vi "Process.vi"(8 "error in":errorcluster, 11 "LHF.SimpleAuth.User":refnum<class "LHF.SimpleAuth.User.lvclass">) -> (0 "error out":errorcluster={"status"=TRUE, "code"=1556, "source"="In Place Element Structure in SMO.lvclass:GetProtectedEvents.vi->SMO.lvclass:Process.vi:5310001->SMO.UI.lvclass:Process.vi:5310001->LHF.SimpleAuth.User.lvclass:Process.vi"}, 3 "LHF.SimpleAuth.User out":refnum<class "LHF.SimpleAuth.User.lvclass">)   [LabVIEW 2013, in "LHF.SimpleAuth.User.lvclass"]
doc: "---------------------------------------------------------------\nJKI State Machine Objects™\nhttp://jki.net/state-machine-objects/\nCopyright (C) 2005-2015, JKI <info@jki.net>\nALL RIGHTS RESERVEDJKI State Machine Objects (SMO) 1.0.0.5\nJKI - JKI\nCopyright (c) 2016, JKI"
uses:
  LHF.SimpleAuth.User.lvclass
  <vilib>/JKI/JKI SMO/SMO/Typedefs/Parent Call--Enum.ctl
  <vilib>/JKI/JKI SMO/SMO.UI/SMO.UI.lvclass
  src/LHF.DB.Mongo.lvclass
  <userlib>/_OpenG.lib/md5/md5.llb/MD5 Message Digest (Hexadecimal String)__ogtk.vi
  <vilib>/JKI/JKI SMO/SMO/SMO.lvclass
panel:
  in  "Action: Edit >> Level":T1(ring)
  in  "Action: Edit >> Name":string
  in  "Action: Edit >> Login":string
  in  "Action: Load User":i32(listbox)=-1
  in  "Action: Search":string
  in  "Action: Save":bool
  in  "Action: Set Password":bool
  in  "Action: Remove":bool
  # "For instructions on how to use the JKI State Machine Objects, examples and video tutorials, visit:\nhttp://jki.net/state-machine-objects/\n\nJKI State Machine Objects™\nhttp://jki.net/state-machine-objects/\nCopyright (C) 2005-2015, JKI <info@jki.net>\nALL RIGHTS RESERVED"
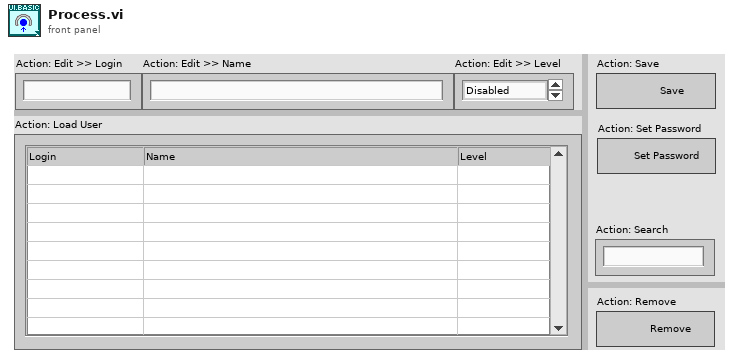
[diagram p1: front panel]
types:
  T1 = enum16{"Disabled", "Operator", "Engineer", "Administrator"}
  T2 = typedef "SMO.lvclass/Parent Call--Enum.ctl" = enum16{"Allows parent to run", "Does not request parent to run"}
  T3 = enum32{"invalid app kind", "Development System", "Run Time System", "Student Edition", "Embedded LabVIEW", "Evaluation", "Custom"}
  T4 = enum32{"Invalid", "Standard", "Closed", "Hidden", "Minimized", "Maximized"}
  T5 = enum32{"Bad", "Idle", "Run top level", "Running"}
  T6 = cluster{"Core":cluster{"Current VI Reference":refnum<vi>, "Close Panel on Exit?":bool, "error":errorcluster}, "Self Reference":refnum<class "LHF.SimpleAuth.User.lvclass">, "Mongo":refnum<class "LHF.DB.Mongo.lvclass">, "_id Array":string[], "_id":string, "User":cluster{"login":string, "name":string, "level":u8}, "Edit":cluster{"login":string, "name":string, "level":u8}}
  T7 = cluster{"login":string, "name":string, "level":u8}
  T8 = cluster{"Current VI Reference":refnum<vi>, "Close Panel on Exit?":bool, "error":errorcluster}
  T9 = typedef "SMO.lvclass/Protected Events.ctl" = cluster{"StopProcesses":refnum<user-event>, "AbortProcesses":refnum<user-event>, "Config Changed":refnum<user-event>}
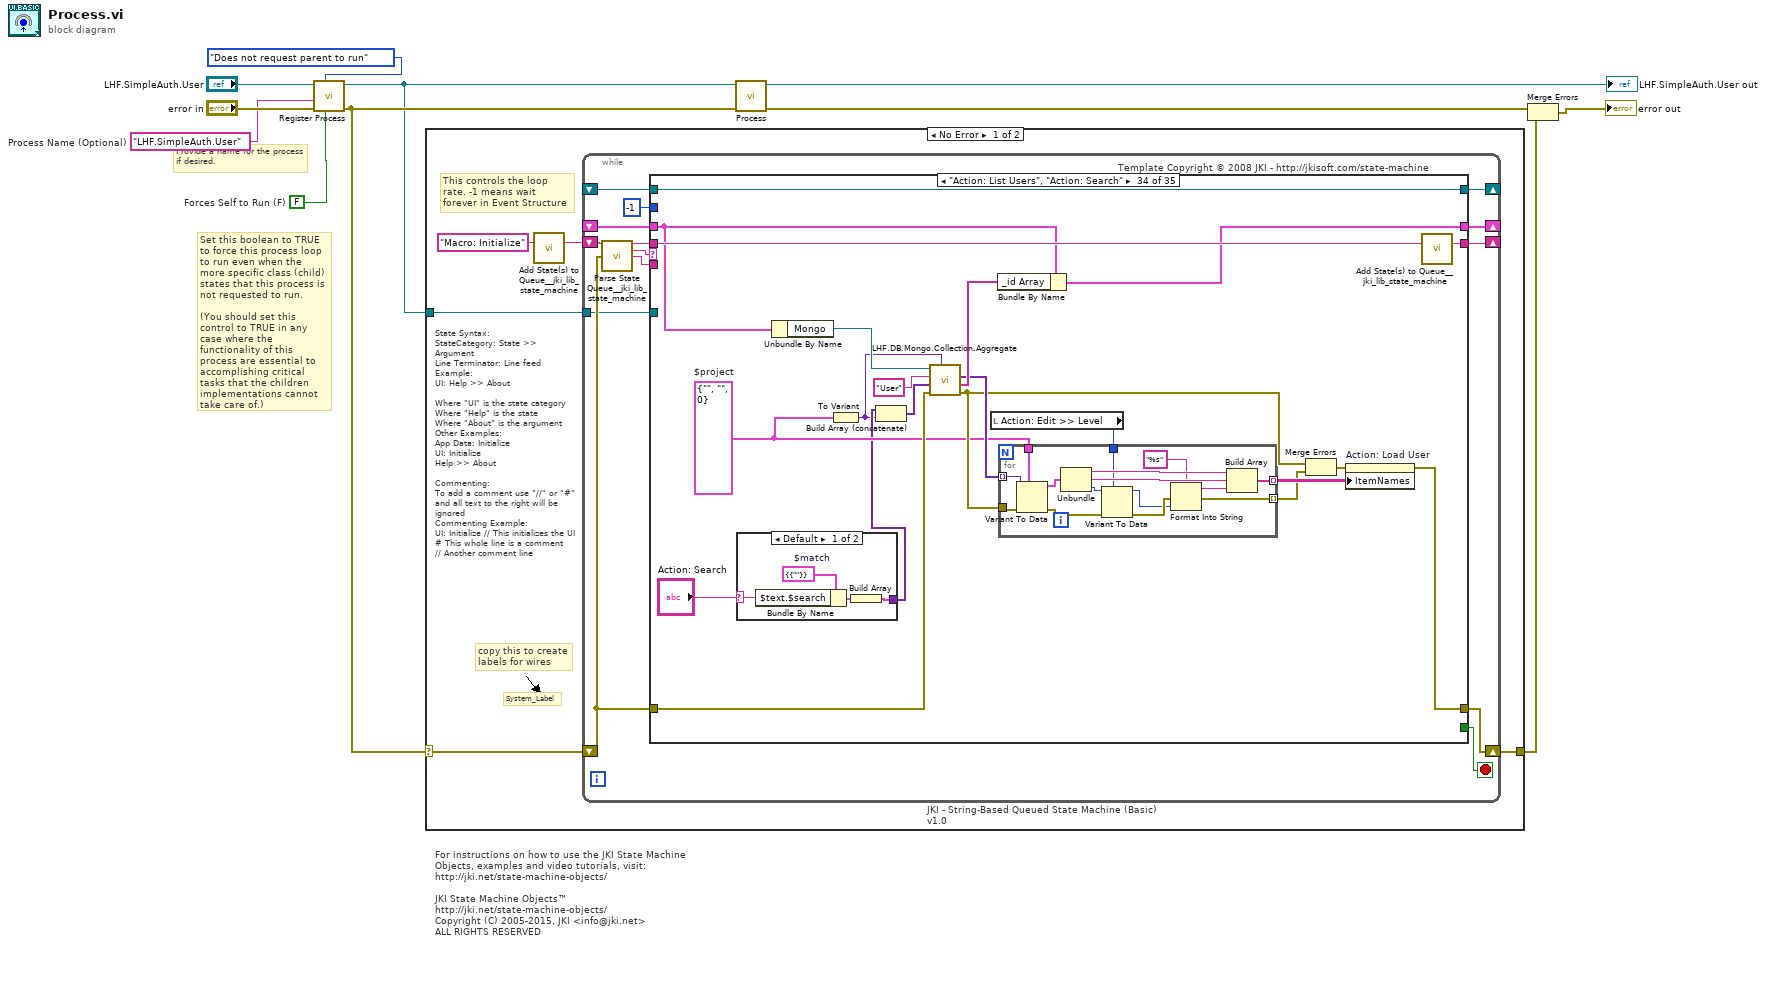
[diagram p0: block diagram]
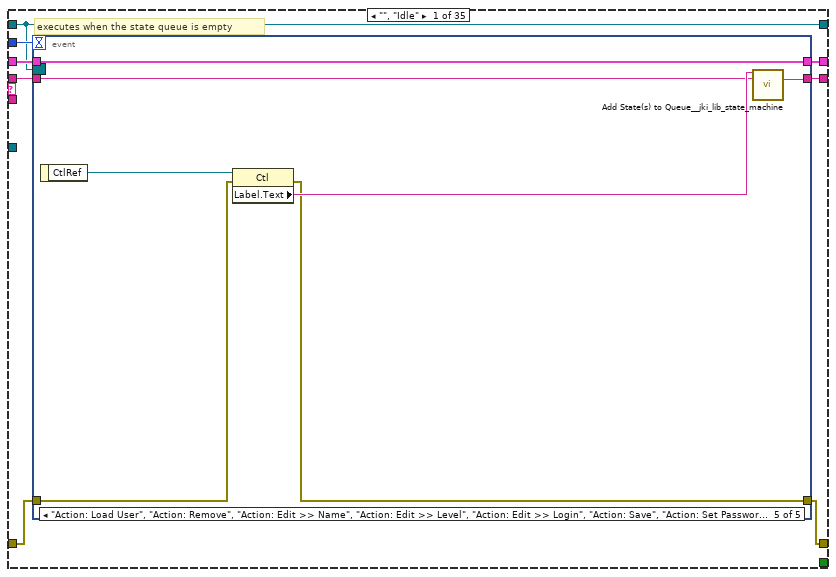
[diagram p2: hidden frame]
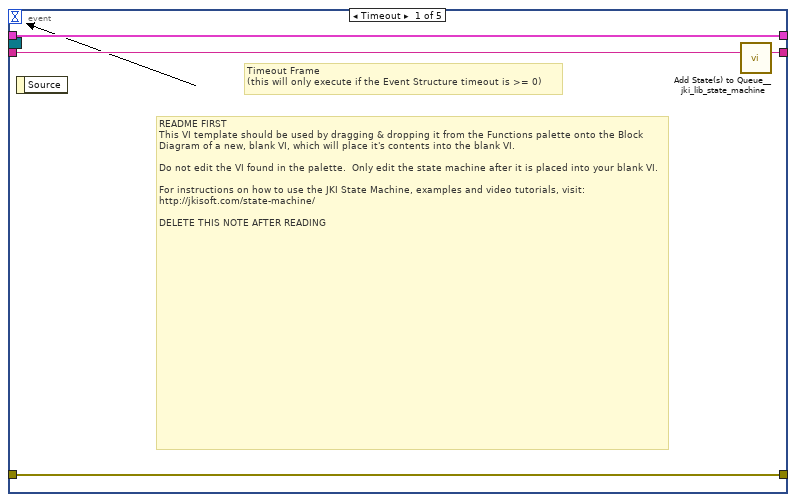
[diagram p3: hidden frame]
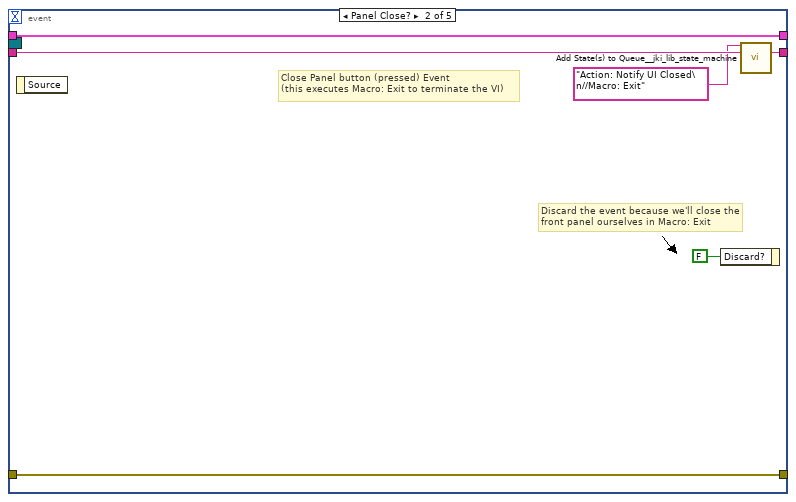
[diagram p4: hidden frame]
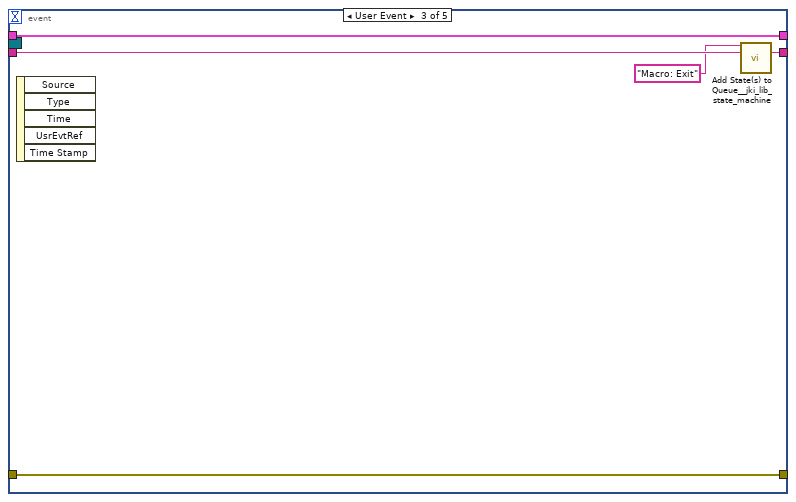
[diagram p5: hidden frame]
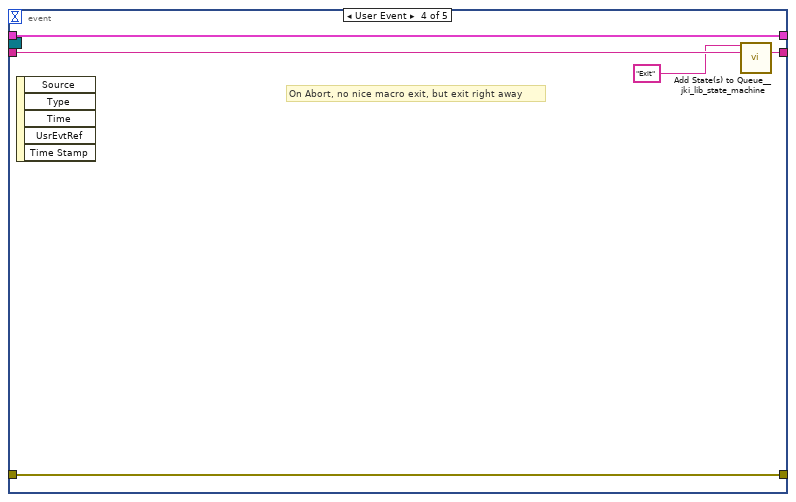
[diagram p6: hidden frame]
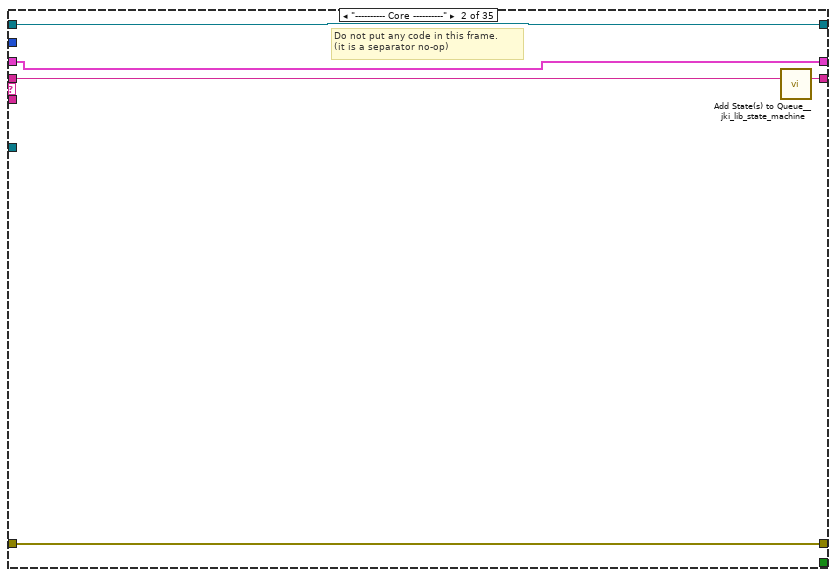
[diagram p7: hidden frame]
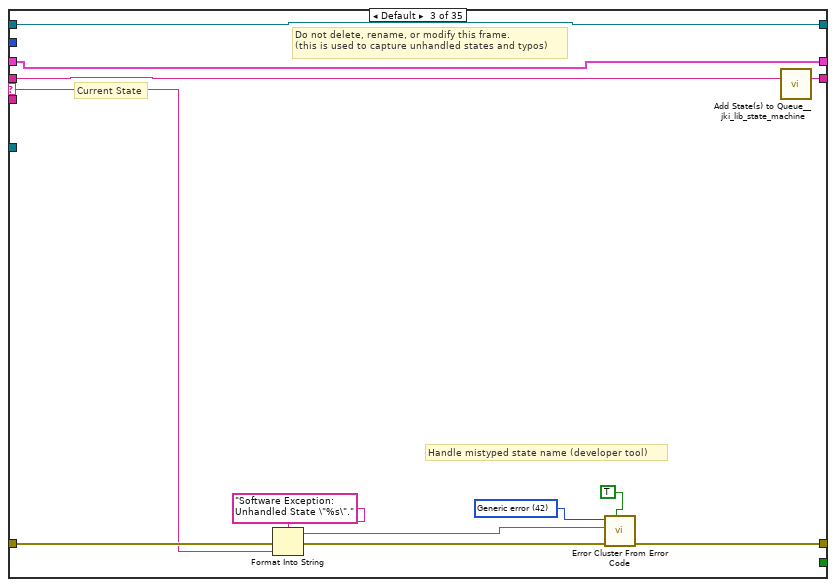
[diagram p8: hidden frame]
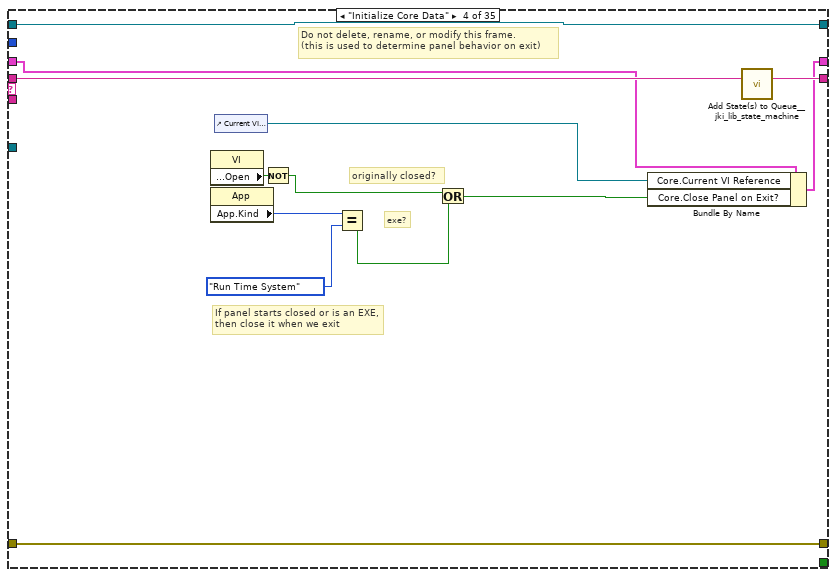
[diagram p9: hidden frame]
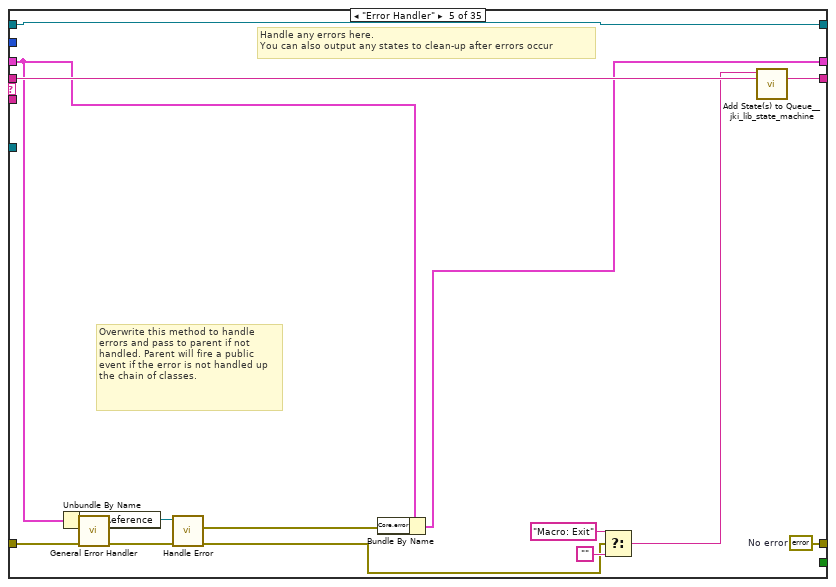
[diagram p10: hidden frame]
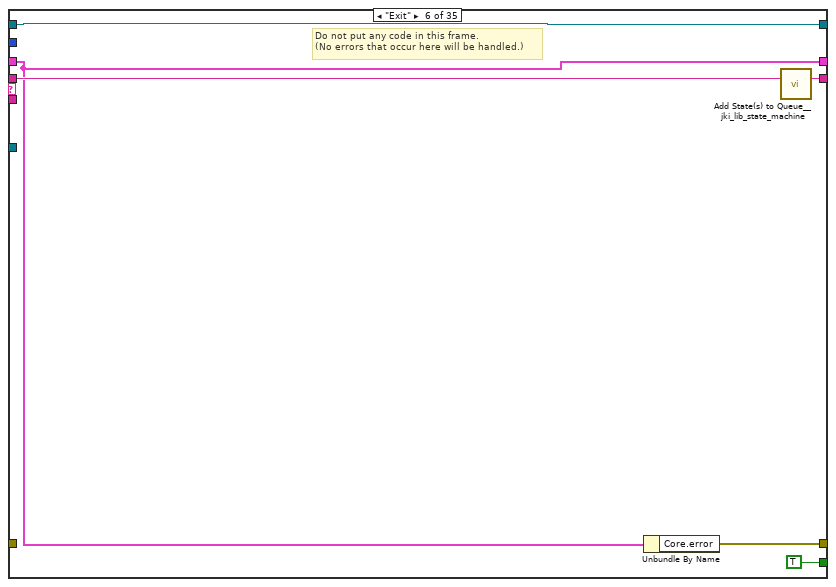
[diagram p11: hidden frame]
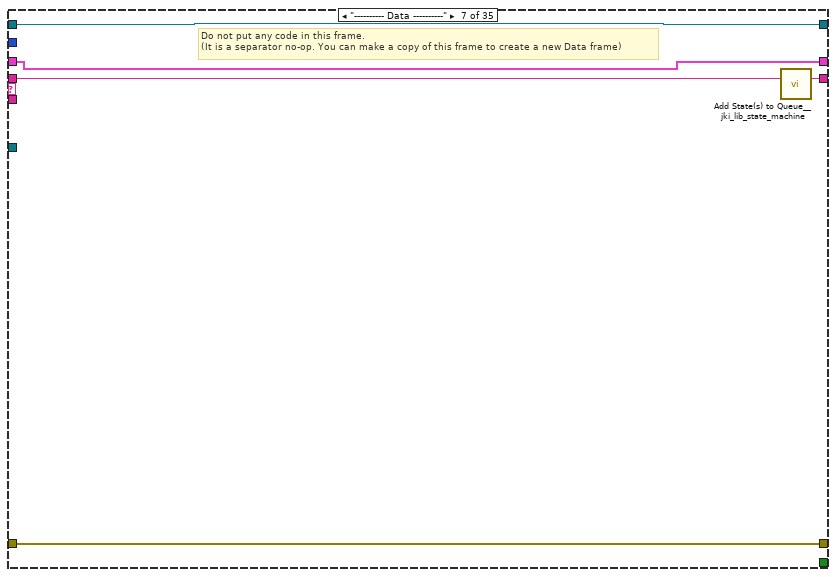
[diagram p12: hidden frame]
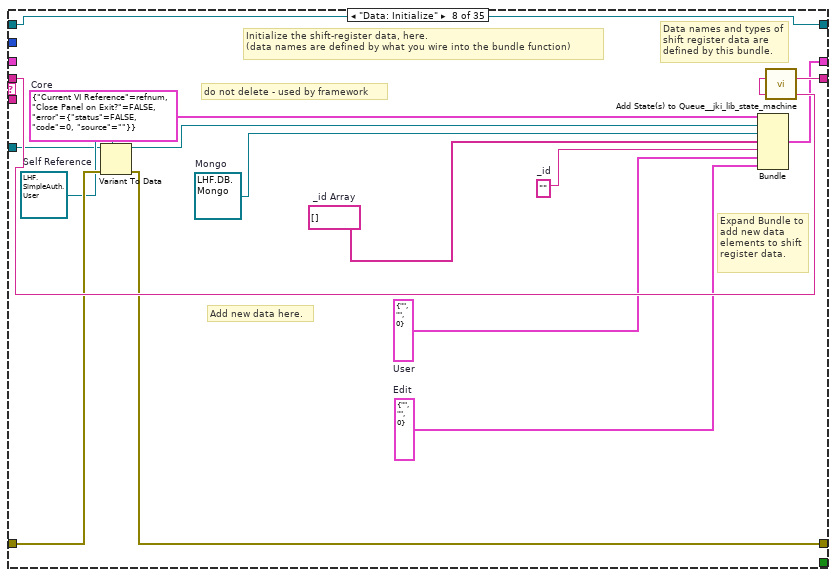
[diagram p13: hidden frame]
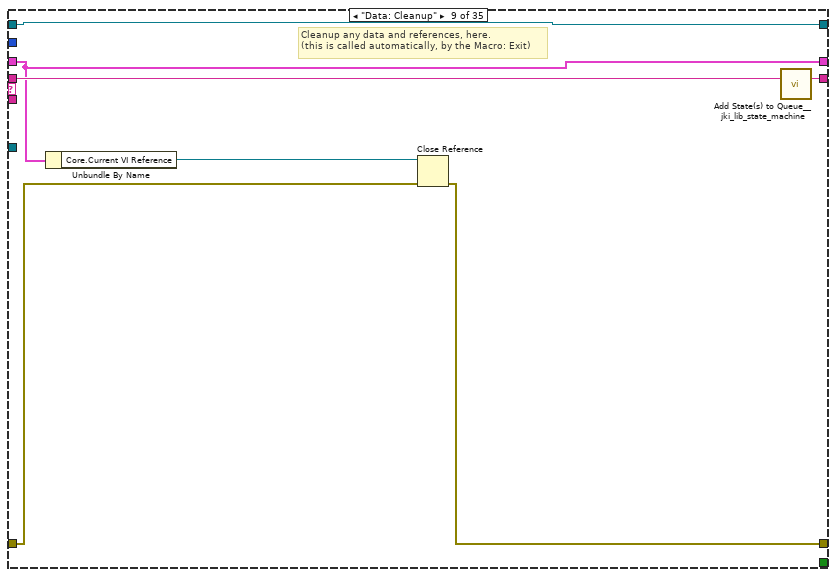
[diagram p14: hidden frame]
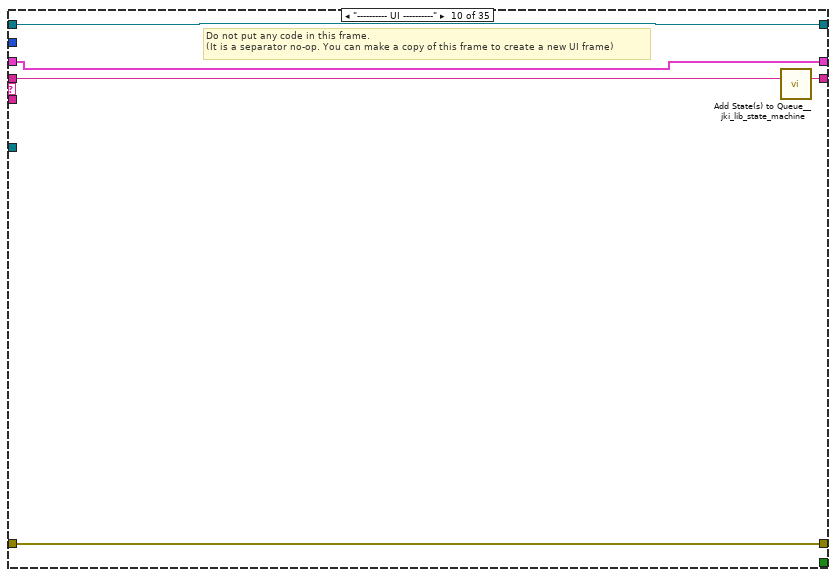
[diagram p15: hidden frame]
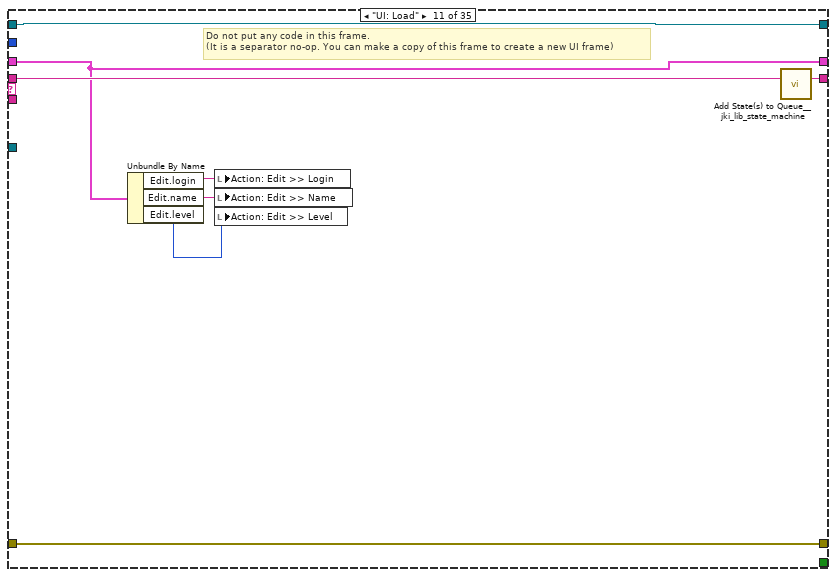
[diagram p16: hidden frame]
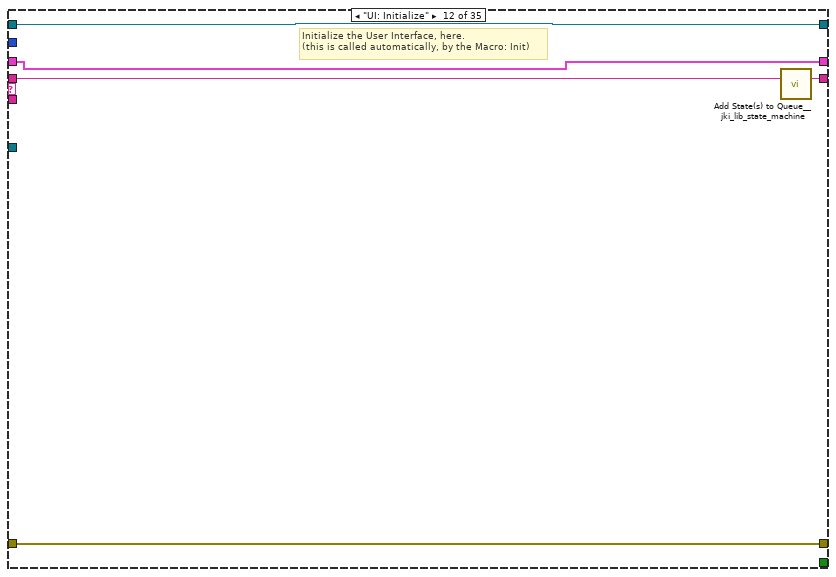
[diagram p17: hidden frame]
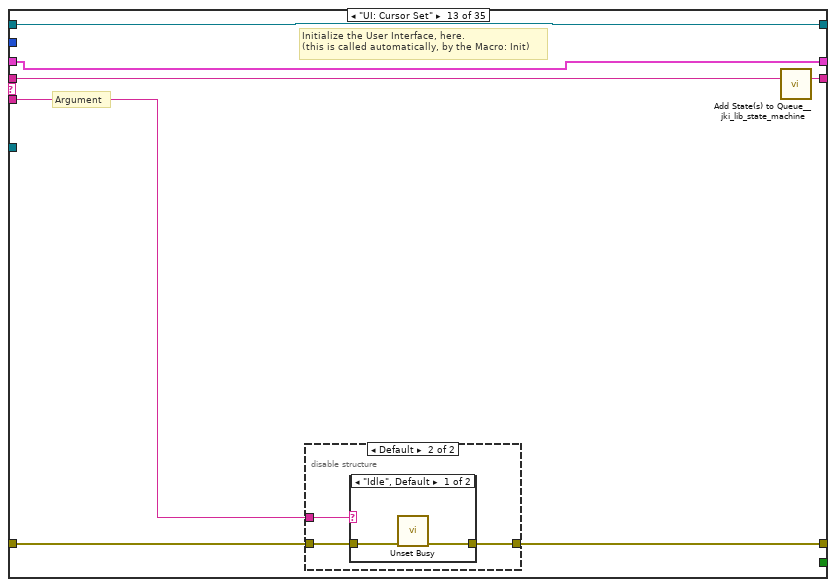
[diagram p18: hidden frame]
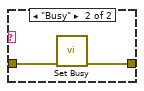
[diagram p20: hidden frame]
diagram:
  w2 = FALSE  # Forces Self to Run (F)
  w1 = "LHF.SimpleAuth.User"  # Process Name (Optional)
  # "Provide a name for the process\nif desired."
  # "Set this boolean to TRUE to force this process loop to run even when the more specific class (child) states that this process is not requested to run.\n\n(You should set this control to TRUE in any case where the functionality of this process are essential to accomplishing critical tasks that the children implementations cannot take care of.)"
  # "For instructions on how to use the JKI State Machine Objects, examples and video tutorials, visit:\nhttp://jki.net/state-machine-objects/\n\nJKI State Machine Objects™\nhttp://jki.net/state-machine-objects/\nCopyright (C) 2005-2015, JKI <info@jki.net>\nALL RIGHTS RESERVED"
  n1 = call <vilib>:"Register Process.vi"("Forces Self to Run (F)"=w2, "Parent Call"=Parent_Call--Enum."Does not request parent to run", "error in (no error)"="error in", "Process Name (optional)"=w1, "SMO"="LHF.SimpleAuth.User") -> ("error out"=w8:errorcluster, "SMO out"=w7:refnum<class "LHF.SimpleAuth.User.lvclass">)  [unwired: 5 in]
  n2 = case shown="No Error" w8 {
    selector: w8 -> [w13 w506]
    tunnel: w7 -> [w14 _]
    tunnel: [w12 w506] -> w4
    frame No Error {
      # "State Syntax:\nStateCategory: State >> Argument\nLine Terminator: Line feed\nExample:\nUI: Help >> About\n\nWhere \"UI\" is the state category\nWhere \"Help\" is the state\nWhere \"About\" is the argument\nOther Examples:\nApp Data: Initialize\nUI: Initialize\nHelp >> About\n\nCommenting:\nTo add a comment use \"//\" or \"#\" and all text to the right will be ignored\nCommenting Example:\nUI: Initialize // This initializes the UI\n# This whole line is a comment\n// Another comment line"
      # "copy this to create labels for wires"
      # "This controls the loop rate. -1 means wait forever in Event Structure"
      # "System_Label"
      n3 = call <vilib>:"Add State(s) to Queue__jki_lib_state_machine.vi"("State(s) in (\"\")"="Macro: Initialize") -> ("States Out"=w16:string)  [unwired: 14 in]
      n4 = while "JKI - String-Based Queued State Machine (Basic) v1.0" {
        shift-right: [w23] -> _
        shift-left: _ -> [w22]
        shift-right: [w26] -> w12
        shift-left: w13 -> [w20]
        shift-right: [w25] -> _
        shift-left: w16 -> [w27]
        tunnel: w14 -> [w19]
        shift-right: [w18] -> _
        shift-left: _ -> [w17]
        stop <- w24 stop-if-true
        # "Template Copyright © 2008 JKI - http://jkisoft.com/state-machine"
        n5 = call <vilib>:"Parse State Queue__jki_lib_state_machine.vi"("State Queue"=w27, "Error In (no error)"=w20) -> ("Remaining States"=w29:string, "Current State"=w30:string, "Arguments"=w28:string)  [unwired: 11 in]
        n6 = case shown="\"Action: List Users\", \"Action: Search\"" w30 {
          selector: w30 -> [_ _ w72 _ _ _ _ _ _ _ _ _ _ _ _ _ _ _ _ _ _ _ _ _ _ _ _ _ _ _ _ _ _ _ _]
          tunnel: w29 -> [w38 w70 w76 w95 w109 w115 w120 w135 w142 w147 w155 w160 w167 w183 w215 w229 w243 w248 w259 w264 w275 w290 w295 w304 w318 w341 w351 w361 w378 w410 w421 w430 w439 w478 w505]
          tunnel: w28 -> [_ _ _ _ _ _ _ _ _ _ _ _ w161 w177 _ _ _ _ _ _ _ _ _ _ _ _ _ _ _ _ _ _ _ _ _]
          tunnel: w22 -> [w36 w67 w74 w86 w98 w111 w117 _ w137 w144 w148 w158 w165 w179 w212 w225 w234 w245 w256 w261 w273 w288 w293 w300 w315 w338 w349 w358 w375 w408 w418 w428 w436 w475 w501]
          tunnel: [w35 w68 w78 w92 w100 w110 w118 w131 w138 w145 w153 w157 w162 w180 w213 w227 w241 w246 w250 w262 w271 w285 w291 w297 w308 w332 w347 w353 w370 w406 w415 w426 w434 w474 w499] -> w26
          tunnel: w20 -> [w34 w68 w77 w92 w105 _ w118 w132 w139 w145 w153 w157 w163 w181 w213 w227 w241 w246 w251 w262 w272 w286 w291 w298 w309 w335 w347 w354 w371 w406 w413 w426 w435 w473 w500]
          tunnel: [w37 w69 w75 w94 w108 w114 w119 w134 w141 w146 w154 w159 w166 w182 w214 w228 w242 w247 w258 w263 w274 w289 w294 w303 w317 w340 w350 w360 w377 w409 w420 w429 w438 w477 w504] -> w25
          tunnel: [_ _ _ _ _ TRUE _ _ _ _ _ _ _ _ _ _ _ _ _ _ _ _ _ _ _ _ _ _ _ _ _ _ _ _ _] -> w24
          tunnel: [w33 w67 w74 w93 w97 w111 w117 w133 w137 w144 w148 w158 w165 w179 w212 w225 w234 w245 w256 w261 w273 w288 w293 w300 w307 w334 w349 w358 w375 w405 w418 w425 w433 w472 w501] -> w23
          tunnel: -1 ("Timeout") -> [w32 _ _ _ _ _ _ _ _ _ _ _ _ _ _ _ _ _ _ _ _ _ _ _ _ _ _ _ _ _ _ _ _ _ _]
          tunnel: w19 -> [_ _ _ _ _ _ _ w129 _ _ _ _ _ _ _ _ _ _ _ _ _ _ _ _ _ _ _ _ _ _ _ _ _ _ _]
          tunnel: [w31 w66 w71 w83 w107 w112 w116 w127 w136 w143 w152 w156 w164 w176 w211 w226 w235 w244 w257 w260 w270 w287 w292 w302 w316 w339 w348 w359 w376 w407 w419 w427 w437 w476 w503] -> w18
          tunnel: w17 -> [w31 w66 w71 w83 w107 w112 w116 w127 w136 w143 w152 w156 w164 w176 w211 w226 w235 w244 w257 w260 w266 w287 w292 w302 w316 w339 w348 w359 w376 w407 w419 w427 w437 w476 w503]
          frame "", "Idle" {
            # "executes when the state queue is empty"
            n7 = event shown="[4] \"Action: Load User\", \"Action: Remove\", \"Action: Edit >> Name\", \"Action: Edit >> Level\", \"Action: Edit >> Login\", \"Action: Save\", \"Action: Set Password\", \"Action: Search\": Value Change" {
              selector: w31 -> [_ _ _ _ _]
              dyn-events: _ -> [_ _ _ _ _]
              timeout: w32 -> [_ _ _ _ _]
              tunnel: w38 -> [w42 w48 w53 w58 w59]
              tunnel: [w41 w47 w52 w57 w64] -> w37
              tunnel: w36 -> [w39 w44 w50 w55 w60]
              tunnel: [w40 w43 w51 w56 w61] -> w35
              tunnel: w34 -> [w40 w43 w51 w56 w62]
              tunnel: [w39 w44 w50 w55 w60] -> w33
              event Timeout {
                # "README FIRST\nThis VI template should be used by dragging & dropping it from the Functions palette onto the Block Diagram of a new, blank VI, which will place it's contents into the blank VI.\n\nDo not edit the VI found in the palette.  Only edit the state machine after it is placed into your blank VI.\n\nFor instructions on how to use the JKI State Machine, examples and video tutorials, visit:\nhttp://jkisoft.com/state-machine/\n\nDELETE THIS NOTE AFTER READING"
                # "Timeout Frame\n(this will only execute if the Event Structure timeout is >= 0)"
                n8 = event-data() -> ()  [unwired: 1 in, 1 out]
                n9 = call <vilib>:"Add State(s) to Queue__jki_lib_state_machine.vi"("State(s) in (\"\")"=w42) -> ("States Out"=w41:string)  [unwired: 14 in]
              }
              event Panel Close? {
                # "Discard the event because we'll close the front panel ourselves in Macro: Exit"
                # "Close Panel button (pressed) Event\n(this executes Macro: Exit to terminate the VI)"
                n10 = event-data() -> ()  [unwired: 1 in, 1 out]
                n11 = event-data("Discard?"=FALSE) -> ()  [unwired: 1 in, 1 out]
                n12 = call <vilib>:"Add State(s) to Queue__jki_lib_state_machine.vi"("State(s) in Front (\"\")"="Action: Notify UI Closed\n//Macro: Exit", "State(s) in (\"\")"=w48) -> ("States Out"=w47:string)  [unwired: 13 in]
              }
              event User Event {
                n13 = event-data() -> ()  [unwired: 1 in, 5 out]
                n14 = call <vilib>:"Add State(s) to Queue__jki_lib_state_machine.vi"("State(s) in Front (\"\")"="Macro: Exit", "State(s) in (\"\")"=w53) -> ("States Out"=w52:string)  [unwired: 13 in]
              }
              event User Event {
                # "On Abort, no nice macro exit, but exit right away"
                n15 = event-data() -> ()  [unwired: 1 in, 5 out]
                n16 = call <vilib>:"Add State(s) to Queue__jki_lib_state_machine.vi"("State(s) in Front (\"\")"="Exit", "State(s) in (\"\")"=w58) -> ("States Out"=w57:string)  [unwired: 13 in]
              }
              event "Action: Load User", "Action: Remove", "Action: Edit >> Name", "Action: Edit >> Level", "Action: Edit >> Login", "Action: Save", "Action: Set Password", "Action: Search": Value Change {
                n17 = event-data() -> ("CtlRef"=w65:refnum<vi>)  [unwired: 1 in]
                n18 = property class="Ctl"(reference=w65, error in=w62) -> (error out=w61:errorcluster, "Label.Text"=w63:string)  [unwired: 1 out]
                n19 = call <vilib>:"Add State(s) to Queue__jki_lib_state_machine.vi"("State(s) in Front (\"\")"=w63, "State(s) in (\"\")"=w59) -> ("States Out"=w64:string)  [unwired: 13 in]
              }
            }
          }
          frame "---------- Core ----------" {
            # "Do not put any code in this frame.\n(it is a separator no-op)"
            n20 = call <vilib>:"Add State(s) to Queue__jki_lib_state_machine.vi"("State(s) in (\"\")"=w70) -> ("States Out"=w69:string)  [unwired: 14 in]
          }
          frame Default {
            w81 = 42 items=["No error", "Argument error", "Memory is full", "Out of zone", "End of file", "File already open", "Generic file I/O error", "File not found", "File permission error", "Disk is full", "Duplicate path", "Too many files open", "System feature not enabled", "Resource file not found", "Cannot add resource", "Resource not found", "Image not found", "Image memory error", "Pen does not exist", "Config type invalid", "Config token not found", "Config parse error", "Config memory error", "Bad external code format", "Bad external code offset", "External code not present", "Null window", "Destroy window error", "Null menu", "Print aborted", "Bad print record", "Print driver error", "Windows error during printing", "Memory error during printing", "Print dialog error", "Generic print error", "Invalid device refnum", "Device not found", "Device parameter error", "Device unit error", "Cannot open device", "Device call aborted", "Generic error", "Cancelled by user", "Object ID too low", "Object ID too high", "Object not in heap", "Unknown heap", "Unknown object (invalid DefProc)", "Unknown object (DefProc not in table)", "Message out of range", "Invalid (null) method", "Unknown message", "Manager call not supported", "Bad address", "Network operation in progress", "Network operation timed out", "Connection is busy", "Network attribute not supported", "Network error", "Address in use", "System out of memory", "Connection aborted", "Connection refused", "Not connected", "Already connected", "Connection closed", "Initialization error (interapplication manager)", "Bad occurrence", "Wait on unbound occurrence handler", "Occurrence queue overflow", "Datalog type conflict", "Unused", "Unrecognized type (interapplication manager)", "Memory corrupt", "Failed to make temporary DLL", "Old CIN version", "Drag socket not found", "Failed to load drop-object", "Failed to register OLE object", "Failed to release OLE object", "Format specifier type mismatch", "Unknown format specifier", "Too few format specifiers", "Too many format specifiers", "Scan failed", "Newer CIN version", "Error converting to variant", "Runtime menu error", "Password tampered", "Variant attribute not found", "Incompatible variant data type", "Event data is not available", "Event Store is not present", "Occurrence is not found", "Event Queue is not created", "Event info is not available", "Refnum passed is NULL", "Error retrieving Class GUID", "Error retrieving CoClass GUID", "Error retrieving TypeLib GUID.", "Bad built application magic bytes.", "Specific driver is different from the specific driver associated with the Logical Name.", "There is no session opened to the class driver.", "Max Error", "MAX - Error with config objects", "MAX - Error loading configuration", "MAX - Group not supported"]
            # "Current State"
            # "Do not delete, rename, or modify this frame.\n(this is used to capture unhandled states and typos)"
            # "Handle mistyped state name (developer tool)"
            n21 = Format Into String(format string="Software Exception: Unhandled State \"%s\"." ("message"), error in=w77, w72) -> (resulting string=w80:string, error out=w79:errorcluster)  [unwired: 1 in]
            n22 = call <vilib>:"Error Cluster From Error Code.vi"("show call chain? (False)"=TRUE, "error in (no error)"=w79, "error message (\"\")"=w80, "error code (0)"=w81) -> ("error out"=w78:errorcluster)  [unwired: 5 in]
            n23 = call <vilib>:"Add State(s) to Queue__jki_lib_state_machine.vi"("State(s) in (\"\")"=w76) -> ("States Out"=w75:string)  [unwired: 14 in]
          }
          frame "Initialize Core Data" {
            # "Do not delete, rename, or modify this frame.\n(this is used to determine panel behavior on exit)"
            # "originally closed?"
            # "exe?"
            # "If panel starts closed or is an EXE, then close it when we exit"
            n24 = property class="VI"() -> ("Front Panel.Open"=w91:bool)  [unwired: 2 in, 2 out]
            n25 = property class="App"() -> ("App.Kind"=w90:T3)  [unwired: 2 in, 2 out]
            n26 = control-ref of="Current VI Reference"() -> (w84:refnum<vi>)
            n27 = Not(x=w91) -> (.not. x?=w88:bool)
            n28 = Equal?(x=w90, y=T3."Run Time System" ("Application:Kind")) -> (x = y?=w87:bool)
            n29 = Or(x=w88, y=w87) -> (x .or. y?=w85:bool)
            n30 = Bundle By Name(cluster=w86, "Core.Current VI Reference"=w84, "Core.Close Panel on Exit?"=w85) -> (w93:T6)
            n31 = call <vilib>:"Add State(s) to Queue__jki_lib_state_machine.vi"("State(s) in (\"\")"=w95) -> ("States Out"=w94:string)  [unwired: 14 in]
          }
          frame "Error Handler" {
            w100 = errorcluster {"status"=FALSE, "code"=0, "source"=""}  # No error
            # "Overwrite this method to handle errors and pass to parent if not handled. Parent will fire a public event if the error is not handled up the chain of classes."
            # "Handle any errors here.\nYou can also output any states to clean-up after errors occur"
            n32 = Unbundle By Name(w98) -> ("Self Reference"=w106:refnum<class "LHF.SimpleAuth.User.lvclass">)
            n33 = call <vilib>:"General Error Handler.vi"("error in (no error)"=w105) -> ("error out"=w96:errorcluster)  [unwired: 10 in, 4 out]
            n34 = call-dynamic "Handle Error.vi"("error in"=w96, "SMO"=w106) -> ("handling error"=w101:errorcluster, "Unhandled error"=w99:errorcluster)  [unwired: 7 in, 1 out]
            n35 = Bundle By Name(cluster=w98, "Core.error"=w99) -> (w97:T6)
            n36 = Select(t="Macro: Exit", s=w101, f="") -> (s? t:f=w102:string)
            n37 = call <vilib>:"Add State(s) to Queue__jki_lib_state_machine.vi"("State(s) in Front (\"\")"=w102, "State(s) in (\"\")"=w109) -> ("States Out"=w108:string)  [unwired: 13 in]
          }
          frame "Exit" {
            # "Do not put any code in this frame.\n(No errors that occur here will be handled.)"
            n38 = Unbundle By Name(w111) -> ("Core.error"=w110:errorcluster)
            n39 = call <vilib>:"Add State(s) to Queue__jki_lib_state_machine.vi"("State(s) in (\"\")"=w115) -> ("States Out"=w114:string)  [unwired: 14 in]
          }
          frame "---------- Data ----------" {
            # "Do not put any code in this frame.\n(It is a separator no-op. You can make a copy of this frame to create a new Data frame)"
            n40 = call <vilib>:"Add State(s) to Queue__jki_lib_state_machine.vi"("State(s) in (\"\")"=w120) -> ("States Out"=w119:string)  [unwired: 14 in]
          }
          frame "Data: Initialize" {
            w121 = ""  # _id
            w122 = T7 {"login"="", "name"="", "level"=0}  # Edit
            w123 = T7 {"login"="", "name"="", "level"=0}  # User
            w124 = string[] []  # _id Array
            w125 = refnum<class "LHF.DB.Mongo.lvclass"> refnum  # Mongo
            w126 = T8 {"Current VI Reference"=refnum, "Close Panel on Exit?"=FALSE, "error"={"status"=FALSE, "code"=0, "source"=""}}  # Core
            w130 = refnum<class "LHF.SimpleAuth.User.lvclass"> refnum  # Self Reference
            # "do not delete - used by framework"
            # "Expand Bundle to add new data elements to shift register data."
            # "Add new data here."
            # "Data names and types of shift register data are defined by this bundle."
            # "Initialize the shift-register data, here.\n(data names are defined by what you wire into the bundle function)"
            n41 = Variant To Data(error in=w132, type=w130, Variant=w129) -> (data=w128:refnum<class "LHF.SimpleAuth.User.lvclass">, error out=w131:errorcluster)
            n42 = Bundle("Core"=w126, "Self Reference"=w128, "Mongo"=w125, "_id Array"=w124, "_id"=w121, "User"=w123, "Edit"=w122) -> (w133:T6)  [unwired: 1 in]
            n43 = call <vilib>:"Add State(s) to Queue__jki_lib_state_machine.vi"("State(s) in (\"\")"=w135) -> ("States Out"=w134:string)  [unwired: 14 in]
          }
          frame "Data: Cleanup" {
            # "Cleanup any data and references, here.\n(this is called automatically, by the Macro: Exit)"
            n44 = Unbundle By Name(w137) -> ("Core.Current VI Reference"=w140:refnum<vi>)
            n45 = Close Reference(reference=w140, error in (no error)=w139) -> (error out=w138:errorcluster)
            n46 = call <vilib>:"Add State(s) to Queue__jki_lib_state_machine.vi"("State(s) in (\"\")"=w142) -> ("States Out"=w141:string)  [unwired: 14 in]
          }
          frame "---------- UI ----------" {
            # "Do not put any code in this frame.\n(It is a separator no-op. You can make a copy of this frame to create a new UI frame)"
            n47 = call <vilib>:"Add State(s) to Queue__jki_lib_state_machine.vi"("State(s) in (\"\")"=w147) -> ("States Out"=w146:string)  [unwired: 14 in]
          }
          frame "UI: Load" {
            # "Do not put any code in this frame.\n(It is a separator no-op. You can make a copy of this frame to create a new UI frame)"
            n48 = Unbundle By Name(w148) -> ("Edit.login"=w151:string, "Edit.name"=w150:string, "Edit.level"=w149:u8)
            n49 = local write "Action: Edit >> Login"(w151) -> ()
            n50 = local write "Action: Edit >> Name"(w150) -> ()
            n51 = local write "Action: Edit >> Level"(w149) -> ()
            n52 = call <vilib>:"Add State(s) to Queue__jki_lib_state_machine.vi"("State(s) in (\"\")"=w155) -> ("States Out"=w154:string)  [unwired: 14 in]
          }
          frame "UI: Initialize" {
            # "Initialize the User Interface, here.\n(this is called automatically, by the Macro: Init)"
            n53 = call <vilib>:"Add State(s) to Queue__jki_lib_state_machine.vi"("State(s) in (\"\")"=w160) -> ("States Out"=w159:string)  [unwired: 14 in]
          }
          frame "UI: Cursor Set" {
            # "Argument"
            # "Initialize the User Interface, here.\n(this is called automatically, by the Macro: Init)"
            n54 = disable-structure shown="Default" {
              disable-tunnel: w163 -> [w168 w171]
              disable-tunnel: [w168 w170] -> w162
              disable-tunnel: w161 -> [_ w169]
              frame condition #0 {
              }
              frame condition #1 (active) {
                n55 = case shown="\"Idle\", Default" w169 {
                  tunnel: w171 -> [w173 w175]
                  tunnel: [w172 w174] -> w170
                  frame "Idle", Default {
                    n56 = call <vilib>:"Unset Busy.vi"("error in (no error)"=w173) -> ("error out"=w172:errorcluster)  [unwired: 10 in]
                  }
                  frame "Busy" {
                    n57 = call <vilib>:"Set Busy.vi"("error in (no error)"=w175) -> ("error out"=w174:errorcluster)  [unwired: 9 in, 1 out]
                  }
                }
              }
            }
            n58 = call <vilib>:"Add State(s) to Queue__jki_lib_state_machine.vi"("State(s) in (\"\")"=w167) -> ("States Out"=w166:string)  [unwired: 14 in]
          }
          frame "UI: Front Panel State" {
            # "Argument"
            # "Set Front Panel Open or Closed\n(Usage: \"UI: Front Panel State >> Open|Close\")"
            n59 = Unbundle By Name(w179) -> ("Core.Current VI Reference"=w178:refnum<vi>)
            n60 = disable-structure shown="Default" {
              disable-tunnel: w181 -> [w187 w210]
              disable-tunnel: [w186 w210] -> w180
              disable-tunnel: w178 -> [w185 _]
              disable-tunnel: w177 -> [w184 _]
              frame condition #0 (active) {
                n61 = case shown="\"Open\", Default" w184 {
                  tunnel: w187 -> [w191 w204]
                  tunnel: [w193 w205] -> w186
                  tunnel: w185 -> [w192 w202]
                  frame "Open", Default {
                    n62 = property class="VI"(reference=w192, error in=w191) -> (reference out=w189:refnum<vi>, error out=w190:errorcluster, "FP.State"=w188:T4)
                    n63 = case shown="\"Closed\"" w188 {
                      tunnel: [w196 w199] -> w193
                      tunnel: w190 -> [w195 w199]
                      tunnel: w189 -> [w194 _]
                      frame "Closed" {
                        n64 = invoke class="VI" method="FP.Open"(reference=w194, error in=w195, "Activate"=TRUE, "State"=T4."Standard") -> (error out=w196:errorcluster)  [unwired: 1 in, 4 out]
                      }
                      frame Default {
                      }
                    }
                  }
                  frame "Close" {
                    n65 = property class="VI"(reference=w202, error in=w204) -> (reference out=w201:refnum<vi>, error out=w203:errorcluster, "FP.State"=w200:T4)
                    n66 = case shown="Default" w200 {
                      tunnel: [w206 w209] -> w205
                      tunnel: w203 -> [w206 w208]
                      tunnel: w201 -> [_ w207]
                      frame "Invalid", "Closed" {
                      }
                      frame Default {
                        n67 = invoke class="VI" method="FP.Close"(reference=w207, error in=w208) -> (error out=w209:errorcluster)  [unwired: 1 in, 2 out]
                      }
                    }
                  }
                }
              }
              frame condition #1 {
              }
            }
            n68 = call <vilib>:"Add State(s) to Queue__jki_lib_state_machine.vi"("State(s) in (\"\")"=w183) -> ("States Out"=w182:string)  [unwired: 14 in]
          }
          frame "---------- Macro ----------" {
            # "Do not put any code in this frame.\n(It is a separator no-op. You can make a copy of this frame to create a new Macro frame)"
            n69 = call <vilib>:"Add State(s) to Queue__jki_lib_state_machine.vi"("State(s) in (\"\")"=w215) -> ("States Out"=w214:string)  [unwired: 14 in]
          }
          frame "Macro: Initialize" {
            w220 = "Database: Connect\nAction: List Users\nUI: Initialize\n//UI: Front Panel State >> Open"  # Database: Connect Action: List Users UI: Initialize //UI: Front Panel State >> Open
            w216 = "Process: Sync"
            # "Initialization Macro\n(This is called once, when the VI starts)"
            n70 = control-ref of="This VI"() -> (w218:refnum<vi>)
            n71 = property class="VI"(reference=w218) -> ("Exec.State"=w217:T5)  [unwired: 1 in, 2 out]
            n72 = Equal?(x=w217, y=T5."Run top level") -> (x = y?=w223:bool)
            n73 = Select(t=w216, s=w223, f="") -> ()  [unwired: 1 out]
            n74 = call <vilib>:"Add State(s) to Queue__jki_lib_state_machine.vi"("State(s) in Front (\"\")"="Data: Initialize\nInitialize Core Data\nEvents: Register\n", "State(s) in (\"\")"=w216, "State(s) at Back (\"\")"=w220) -> ("States Out"=w219:string)  [unwired: 12 in]
            n75 = call <vilib>:"Add State(s) to Queue__jki_lib_state_machine.vi"("State(s) in Front (\"\")"=w219, "State(s) in (\"\")"=w229) -> ("States Out"=w228:string)  [unwired: 13 in]
          }
          frame "Macro: Exit" {
            # "Exit Macro\n(This is called once, when the VI exits)"
            n76 = Unbundle By Name(w234) -> ("Core.Close Panel on Exit?"=w240:bool)
            n77 = Select(t="//UI: Front Panel State >> Close", s=w240, f="") -> (s? t:f=w237:string)
            n78 = call <vilib>:"Add State(s) to Queue__jki_lib_state_machine.vi"("State(s) in Front (\"\")"="Data: Cleanup\nEvents: Unregister\nDatabase: Disconnect", "State(s) in (\"\")"="Process: Sync", "State(s) at Back (\"\")"="Exit") -> ("States Out"=w231:string)  [unwired: 12 in]
            n79 = call <vilib>:"Add State(s) to Queue__jki_lib_state_machine.vi"("State(s) in (\"\")"=w237, "State(s) at Back (\"\")"=w231) -> ("States Out"=w236:string)  [unwired: 13 in]
            n80 = call <vilib>:"Add State(s) to Queue__jki_lib_state_machine.vi"("State(s) in Front (\"\")"=w236, "State(s) in (\"\")"=w243) -> ("States Out"=w242:string)  [unwired: 13 in]
          }
          frame "---------- Process ----------" {
            # "Template Separator\n(You can make a copy of, or modify, this frame)"
            n81 = call <vilib>:"Add State(s) to Queue__jki_lib_state_machine.vi"("State(s) in (\"\")"=w248) -> ("States Out"=w247:string)  [unwired: 14 in]
          }
          frame "Process: Sync" {
            n82 = Unbundle By Name(w256) -> ("Self Reference"=w252:refnum<class "LHF.SimpleAuth.User.lvclass">)
            n83 = call <vilib>:"WaitOnProcessSync.vi"("error in (no error)"=w251, "SMO"=w252) -> ("error out"=w250:errorcluster, "Don't run?"=w255:bool)  [unwired: 7 in, 1 out]
            n84 = Select(t="Data: Cleanup\nEvents: Unregister\nExit", s=w255, f="") -> (s? t:f=w249:string)
            n85 = call <vilib>:"Add State(s) to Queue__jki_lib_state_machine.vi"("State(s) in Front (\"\")"=w249, "State(s) in (\"\")"=w259) -> ("States Out"=w258:string)  [unwired: 13 in]
          }
          frame "---------- Events ----------" {
            # "Template Separator\n(You can make a copy of, or modify, this frame)"
            n86 = call <vilib>:"Add State(s) to Queue__jki_lib_state_machine.vi"("State(s) in (\"\")"=w264) -> ("States Out"=w263:string)  [unwired: 14 in]
          }
          frame "Events: Register" {
            # "Self Events (API Calls)"
            # "Base Class Protected Events"
            n87 = Unbundle By Name(w273) -> ("Self Reference"=w268:refnum<class "LHF.SimpleAuth.User.lvclass">)
            n88 = call <vilib>:"GetProtectedEvents.vi"("error in (no error)"=w272, "SMO"=w268) -> ("error out"=w265:errorcluster, "SMO Protected Events"=w269:T9)  [unwired: 7 in, 1 out]
            n89 = Not A Number/Path/Refnum?(number/path/refnum=w266) -> (NaN/Path/Refnum?=w267:bool)
            n90 = case shown="False" w267 {
              tunnel: [w279 w284] -> w271
              tunnel: [w278 w283] -> w270
              tunnel: w269 -> [w277 w282]
              tunnel: w265 -> [w276 w281]
              tunnel: w266 -> [_ w280]
              frame True {
                # "Expand to add\nmore events"
                n91 = register-events(error in=w276, w277) -> (reference out=w278:refnum<event-registration>, error out=w279:errorcluster)  [unwired: 1 in]
              }
              frame False {
                n92 = register-events(reference=w280, error in=w281, w282) -> (reference out=w283:refnum<event-registration>, error out=w284:errorcluster)
              }
            }
            n93 = call <vilib>:"Add State(s) to Queue__jki_lib_state_machine.vi"("State(s) in (\"\")"=w275) -> ("States Out"=w274:string)  [unwired: 14 in]
          }
          frame "Events: Unregister" {
            n94 = Unregister For Events(event registration refnum=w287, error in=w286) -> (error out=w285:errorcluster)
            n95 = call <vilib>:"Add State(s) to Queue__jki_lib_state_machine.vi"("State(s) in (\"\")"=w290) -> ("States Out"=w289:string)  [unwired: 14 in]
          }
          frame "---------- Database ----------" {
            n96 = call <vilib>:"Add State(s) to Queue__jki_lib_state_machine.vi"("State(s) in (\"\")"=w295) -> ("States Out"=w294:string)  [unwired: 14 in]
          }
          frame "Database: Setup" {
            w296 = "text"  # name
            n97 = Unbundle By Name(w300) -> ("Mongo"=w299:refnum<class "LHF.DB.Mongo.lvclass">)
            n98 = call-dynamic "LHF.DB.Mongo.Collection.EnsureIndex.vi"("error in (no error)"=w298, "value"=w296, "Collection"="User", "LHF.DB.Mongo in"=w299) -> ("error out"=w297:errorcluster)  [unwired: 6 in, 1 out]
            n99 = call <vilib>:"Add State(s) to Queue__jki_lib_state_machine.vi"("State(s) in (\"\")"=w304) -> ("States Out"=w303:string)  [unwired: 14 in]
          }
          frame "Database: Connect" {
            w310 = "Example" ("database")
            w311 = "mongodb://localhost/" ("url")
            n100 = Unbundle By Name(w315) -> ("Mongo"=w314:refnum<class "LHF.DB.Mongo.lvclass">)
            n101 = call-dynamic "LHF.DB.Mongo.Client.Connect.vi"("error in (no error)"=w309, "database"=w310, "url"=w311, "LHF.DB.Mongo in"=w314) -> ("error out"=w312:errorcluster, "LHF.DB.Mongo out"=w313:refnum<class "LHF.DB.Mongo.lvclass">)  [unwired: 6 in]
            n102 = case shown="No Error" w312 {
              selector: w312 -> [w319 _]
              tunnel: w313 -> [w320 w330]
              tunnel: w311 -> [_ w328]
              tunnel: w310 -> [_ w327]
              tunnel: [w320 w325] -> w306
              tunnel: [w319 w324] -> w308
              frame No Error {
              }
              frame Error {
                n103 = call <vilib>:"Application Directory.vi"() -> ("Application Directory"=w323:path)
                n104 = Build Path(base path=w323, name or relative path="data\\db") -> (appended path=w322:path)
                n105 = call-dynamic "LHF.DB.Mongo.Daemon.Start.vi"("data folder"=w322, "mongod path"=path "C:/Program Files/MongoDB/Server/3.2/bin/mongod.exe", "LHF.DB.Mongo in"=w330) -> ("error out"=w326:errorcluster, "LHF.DB.Mongo out"=w329:refnum<class "LHF.DB.Mongo.lvclass">)  [unwired: 7 in]
                n106 = call-dynamic "LHF.DB.Mongo.Client.Connect.vi"("error in (no error)"=w326, "database"=w327, "url"=w328, "LHF.DB.Mongo in"=w329) -> ("error out"=w324:errorcluster, "LHF.DB.Mongo out"=w325:refnum<class "LHF.DB.Mongo.lvclass">)  [unwired: 6 in]
              }
            }
            n107 = Bundle By Name(cluster=w315, "Mongo"=w306) -> (w307:T6)
            n108 = call <vilib>:"Add State(s) to Queue__jki_lib_state_machine.vi"("State(s) in Front (\"\")"="Database: Setup" ("State(s) in Front (\"\")"), "State(s) in (\"\")"=w318) -> ("States Out"=w317:string)  [unwired: 13 in]
          }
          frame "Database: Disconnect" {
            n109 = Unbundle By Name(w338) -> ("Mongo"=w337:refnum<class "LHF.DB.Mongo.lvclass">)
            n110 = call-dynamic "LHF.DB.Mongo.Client.Disconnect.vi"("error in (no error)"=w335, "LHF.DB.Mongo in"=w337) -> ("error out"=w332:errorcluster, "LHF.DB.Mongo out"=w336:refnum<class "LHF.DB.Mongo.lvclass">)  [unwired: 8 in]
            n111 = disable-structure shown="Enabled" {
              disable-tunnel: w336 -> [w345 w346]
              disable-tunnel: [w343 w346] -> w333
              disable-tunnel: w332 -> [w342 _]
              frame Disabled {
                n112 = call-dynamic "LHF.DB.Mongo.Daemon.Shutdown.vi"("error in (no error)"=w342, "LHF.DB.Mongo in"=w345) -> ("error out"=w344:errorcluster, "LHF.DB.Mongo out"=w343:refnum<class "LHF.DB.Mongo.lvclass">)  [unwired: 8 in]
                n113 = call <vilib>:"Clear Errors.vi"("error in (no error)"=w344) -> ()  [unwired: 6 in, 1 out]
              }
              frame Enabled {
              }
            }
            n114 = Bundle By Name(cluster=w338, "Mongo"=w333) -> (w334:T6)
            n115 = call <vilib>:"Add State(s) to Queue__jki_lib_state_machine.vi"("State(s) in (\"\")"=w341) -> ("States Out"=w340:string)  [unwired: 14 in]
          }
          frame "---------- Action ----------" {
            n116 = call <vilib>:"Add State(s) to Queue__jki_lib_state_machine.vi"("State(s) in (\"\")"=w351) -> ("States Out"=w350:string)  [unwired: 14 in]
          }
          frame "Action: Remove" {
            n117 = local read "Action: Load User"() -> (w357:i32)
            n118 = Unbundle By Name(w358) -> ("Mongo"=w355:refnum<class "LHF.DB.Mongo.lvclass">, "_id Array"=w356:string[])
            n119 = case shown="0.." w357 {
              selector: w357 -> [_ w368]
              tunnel: w356 -> [_ w369]
              tunnel: w355 -> [_ w367]
              tunnel: w354 -> [w362 w365]
              tunnel: [w362 w364] -> w353
              frame Default {
              }
              frame 0.. {
                n120 = Index Array(array=w369, index=w368) -> (element=w363:string)
                n121 = call-dynamic "LHF.DB.Mongo.Collection.RemoveById.vi"("error in (no error)"=w365, "_id"=w363, "collectionName"="User", "LHF.DB.Mongo in"=w367) -> ("error out"=w364:errorcluster)  [unwired: 6 in, 1 out]
              }
            }
            n122 = call <vilib>:"Add State(s) to Queue__jki_lib_state_machine.vi"("State(s) in Front (\"\")"="Action: Clear\nAction: List Users" ("State(s) in Front (\"\")"), "State(s) in (\"\")"=w361) -> ("States Out"=w360:string)  [unwired: 13 in]
          }
          frame "Action: Set Password" {
            n123 = local read "Action: Load User"() -> (w373:i32)
            n124 = Unbundle By Name(w375) -> ("Mongo"=w372:refnum<class "LHF.DB.Mongo.lvclass">, "_id Array"=w374:string[])
            n125 = case shown="0.." w373 {
              selector: w373 -> [_ w386]
              tunnel: w374 -> [_ w388]
              tunnel: w372 -> [_ w384]
              tunnel: w371 -> [w379 w381]
              tunnel: [w379 w380] -> w370
              frame Default {
              }
              frame 0.. {
                n126 = call "Prompt User for Input"("error in (no error)"=w381) -> ("Password"=w385:string, "OK"=w387:bool, "error out"=w382:errorcluster)  [unwired: 16 in]
                n127 = Index Array(array=w388, index=w386) -> (element=w383:string)
                n128 = case shown="True" w387 {
                  tunnel: w385 -> [_ w400]
                  tunnel: w384 -> [_ w399]
                  tunnel: w383 -> [_ w396]
                  tunnel: w382 -> [w389 w398]
                  tunnel: [w389 w397] -> w380
                  frame False {
                  }
                  frame True {
                    w392 = ""  # password
                    w395 = ""  # _id
                    n129 = call-poly <userlib>:"MD5 Message Digest__ogtk.vi"("Message"=w400) -> ("MD5 Message Digest"=w393:string)
                    n130 = Variant To Data(type=w395, Variant=w396) -> (data=w390:string)  [unwired: 1 in, 1 out]
                    n131 = Variant To Data(type=w392, Variant=w393) -> (data=w391:string)  [unwired: 1 in, 1 out]
                    n132 = call-dynamic "LHF.DB.Mongo.Collection.Update.vi"("Query"=w390, "error in (no error)"=w398, "Update"=w391, "Collection"="User", "LHF.DB.Mongo in"=w399) -> ("error out"=w397:errorcluster)  [unwired: 3 in, 3 out]
                  }
                }
              }
            }
            n133 = call <vilib>:"Add State(s) to Queue__jki_lib_state_machine.vi"("State(s) in (\"\")"=w378) -> ("States Out"=w377:string)  [unwired: 14 in]
          }
          frame "Action: Clear" {
            w401 = ""  # _id
            w404 = T7 {"login"="", "name"="", "level"=0} ("User")
            n134 = Bundle By Name(cluster=w408, "User"=w404, "Edit"=w404, "_id"=w401) -> (w405:T6)
            n135 = property on="Action: Load User" class="MCListbox (strict)"("Value"=-1 ("Action: Load User")) -> ()  [unwired: 2 in, 2 out]
            n136 = call <vilib>:"Add State(s) to Queue__jki_lib_state_machine.vi"("State(s) in Front (\"\")"="UI: Load" ("State(s) in Front (\"\")"), "State(s) in (\"\")"=w410) -> ("States Out"=w409:string)  [unwired: 13 in]
          }
          frame "Action: Save" {
            n137 = Unbundle By Name(w418) -> ("Mongo"=w416:refnum<class "LHF.DB.Mongo.lvclass">, "_id"=w412:string, "Edit"=w411:T7)
            n138 = call-dynamic "LHF.DB.Mongo.Collection.Insert.vi"("Document"=w411, "error in (no error)"=w413, "_id"=w412, "Collection"="User", "LHF.DB.Mongo"=w416) -> ("error out"=w415:errorcluster)  [unwired: 3 in, 3 out]
            n139 = call <vilib>:"Add State(s) to Queue__jki_lib_state_machine.vi"("State(s) in Front (\"\")"="Action: Clear\nAction: List Users" ("State(s) at Back (\"\")"), "State(s) in (\"\")"=w421) -> ("States Out"=w420:string)  [unwired: 13 in]
          }
          frame "Action: Edit" {
            n140 = Bundle By Name(cluster=w428, "Edit.login"="Action: Edit >> Login", "Edit.name"="Action: Edit >> Name", "Edit.level"="Action: Edit >> Level") -> (w425:T6)
            n141 = call <vilib>:"Add State(s) to Queue__jki_lib_state_machine.vi"("State(s) in (\"\")"=w430) -> ("States Out"=w429:string)  [unwired: 14 in]
          }
          frame "Action: Load User" {
            n142 = case shown="0.." "Action: Load User" {
              selector: "Action: Load User" -> [_ w452]
              tunnel: w436 -> [w442 w457]
              tunnel: w435 -> [w440 w454]
              tunnel: [w440 w444] -> w434
              tunnel: [w442 w453] -> w433
              tunnel: ["Action: Clear" "UI: Load"] -> w431
              frame ..-1 {
              }
              frame 0.. {
                n143 = Unbundle By Name(w457) -> ("User"=w445:T7, "_id Array"=w451:string[], "Mongo"=w456:refnum<class "LHF.DB.Mongo.lvclass">)
                n144 = Index Array(array=w451, index=w452) -> (element=w449:string)
                n145 = call-dynamic "LHF.DB.Mongo.Util.GetDocumentPart.vi"("projection type"=w445, "error in (no error)"=w454, "_id"=w449, "Collection"="User", "LHF.DB.Mongo in"=w456) -> ("error out"=w448:errorcluster, "_id"=w446:string, "Document"=w447:variant)  [unwired: 3 in, 1 out]
                n146 = Variant To Data(error in=w448, type=w445, Variant=w447) -> (data=w443:T7, error out=w444:errorcluster)
                n147 = Bundle By Name(cluster=w457, "_id"=w446, "User"=w443, "Edit"=w443) -> (w453:T6)
              }
            }
            n148 = call <vilib>:"Add State(s) to Queue__jki_lib_state_machine.vi"("State(s) in Front (\"\")"=w431, "State(s) in (\"\")"=w439) -> ("States Out"=w438:string)  [unwired: 13 in]
          }
          frame "Action: List Users", "Action: Search" {
            w461 = T7 {"login"="", "name"="", "level"=0}  # $project
            n149 = case shown="Default" "Action: Search" {
              selector: "Action: Search" -> [w496 _]
              tunnel: [w494 variant[] [] ("appended array")] -> w459
              frame Default {
                w497 = cluster{"$text":cluster{"$search":string}} {"$text"={"$search"=""}}  # $match
                n150 = Bundle By Name(cluster=w497, "$text.$search"=w496) -> (w495:cluster{"$text":cluster{"$search":string}})
                n151 = Build Array(w495) -> (w494:cluster{"$text":cluster{"$search":string}}[])
              }
              frame "" {
              }
            }
            n152 = Unbundle By Name(w475) -> ("Mongo"=w470:refnum<class "LHF.DB.Mongo.lvclass">)
            n153 = To Variant(anything=w461) -> (Variant=w458:variant)
            n154 = Build Array (concatenate)(w459, w458) -> (w462:variant[])
            n155 = call-dynamic "LHF.DB.Mongo.Collection.Aggregate.vi"("return type"=w458, "error in (no error)"=w473, "Operations"=w462, "Collection"="User", "LHF.DB.Mongo in"=w470) -> ("error out"=w464:errorcluster, "_id Array"=w471:string[], "Documents"=w469:variant[])  [unwired: 3 in, 1 out]
            n156 = local read "Action: Edit >> Level"() -> (w468:T1)
            n157 = Bundle By Name(cluster=w475, "_id Array"=w471) -> (w472:T6)
            n158 = for {
              tunnel: w469 -> [w483] mode=indexing
              tunnel: w468 -> [w490]
              tunnel: [w485] -> w467 mode=indexing
              tunnel: [w484] -> w466 mode=indexing
              tunnel: w464 -> [w480]
              tunnel: w461 -> [w479]
              n159 = Variant To Data(error in=w480, type=w479, Variant=w483) -> (data=w482:T7, error out=w481:errorcluster)
              n160 = Unbundle(w482) -> ("login"=w493:string, "name"=w492:string, "level"=w491:u8)
              n161 = Variant To Data(error in=w481, type=w490, Variant=w491) -> (data=w488:T1, error out=w489:errorcluster)
              n162 = Format Into String(format string="%s", error in=w489, w488) -> (resulting string=w486:string, error out=w484:errorcluster)  [unwired: 1 in]
              n163 = Build Array(w493, w492, w486) -> (w485:string[])
            }
            n164 = Merge Errors(w464, w466) -> (w465:errorcluster)
            n165 = property on="Action: Load User" class="MCListbox (strict)"(error in=w465, "ItemNames"=w467) -> (error out=w474:errorcluster)  [unwired: 1 in, 1 out]
            n166 = call <vilib>:"Add State(s) to Queue__jki_lib_state_machine.vi"("State(s) in (\"\")"=w478) -> ("States Out"=w477:string)  [unwired: 14 in]
          }
          frame "Action: Notify UI Closed" {
            # "Notify that the UI has been closed"
            n167 = Unbundle By Name(w501) -> ("Self Reference"=w502:refnum<class "LHF.SimpleAuth.User.lvclass">)
            n168 = call <vilib>:"Hide.vi"("error in (no error)"=w500, "SMO.UI"=w502) -> ("error out"=w499:errorcluster)  [unwired: 8 in, 1 out]
            n169 = call <vilib>:"Add State(s) to Queue__jki_lib_state_machine.vi"("State(s) in (\"\")"=w505) -> ("States Out"=w504:string)  [unwired: 14 in]
          }
        }
      }
    }
    frame Error {
    }
  }
  n170 = call-parent "Process.vi"("error in (no error)"=w8, "SMO.UI"=w7) -> ("error out"=w5:errorcluster, "SMO.UI out"=→"LHF.SimpleAuth.User out":refnum<class "LHF.SimpleAuth.User.lvclass">)  [unwired: 8 in]
  n171 = Merge Errors(w5, w4) -> (→"error out":errorcluster)
